vi "Tree_FocusArrayPath_Tests.vi"(11 "error in":errorcluster) -> (15 "error out":errorcluster)   [LabVIEW 2016, in "DronaTest.lvlib"]
uses:
  DronaTest.lvlib
  APIs/Stimulus/ControlValue/SetValueAuto.vi
  APIs/Stimulus/ControlValue/Controls/Tree/SetValueByHierarchicalPathArray.vi
  APIs/Assert/AssertControlValue/Controls/Tree/AssertValueByArrayPath.vi
  <vilib>/addons/_JKI Toolkits/Caraya/classes/Assert/Assert Error.vi
  <vilib>/addons/_JKI Toolkits/Caraya/classes/Assert/Assert Equal Value_Variant.vi
  <vilib>/addons/_JKI Toolkits/Caraya/classes/Test/Test.lvclass
  Drona.lvlib
  <vilib>/SLL Toolkit/SLL Debug/SLL Debug.lvlib
  <vilib>/addons/_JKI Toolkits/Caraya/classes/Assert/Assert.lvclass
  APIs/Stimulus/ControlValue/Controls/Tree/StimulusTree.lvlib
  APIs/Assert/AssertControlValue/Controls/Tree/AssertTree.lvlib
  APIs/Stimulus/ControlValue/ControlValue.lvlib
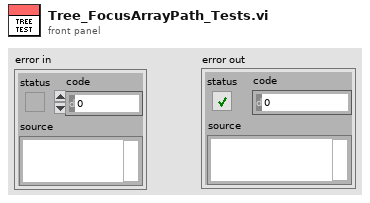
[diagram p1: front panel]
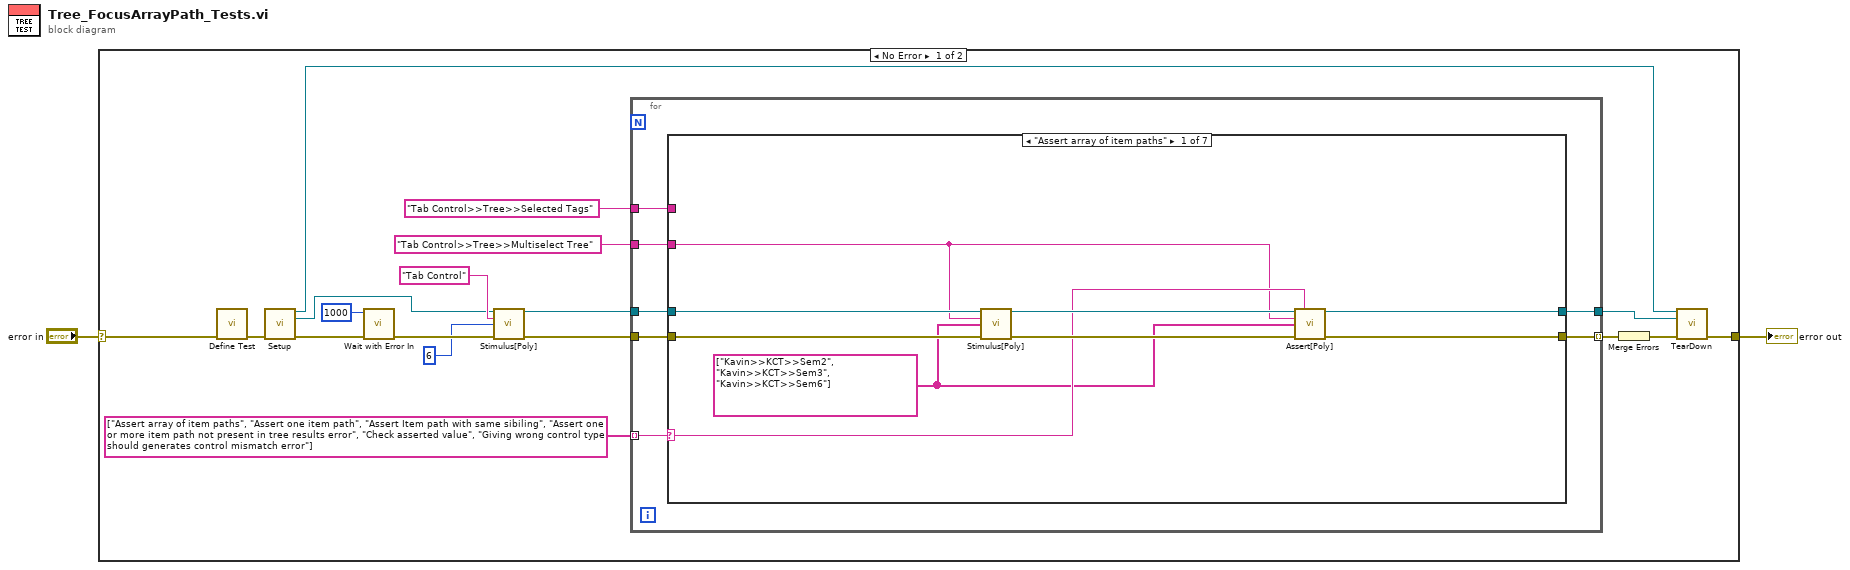
[diagram p0: block diagram]
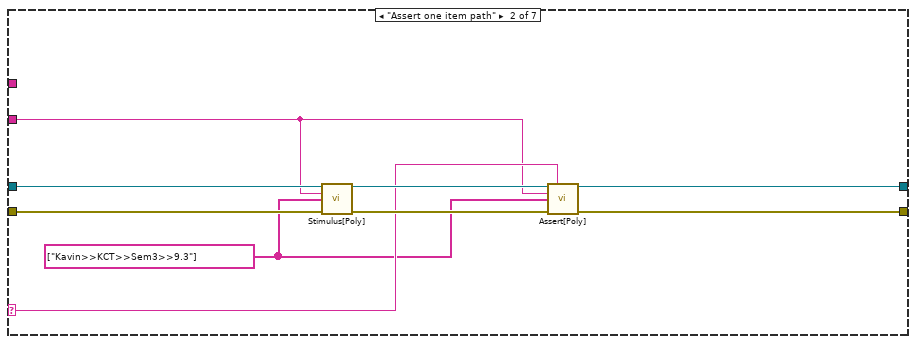
[diagram p2: hidden frame]
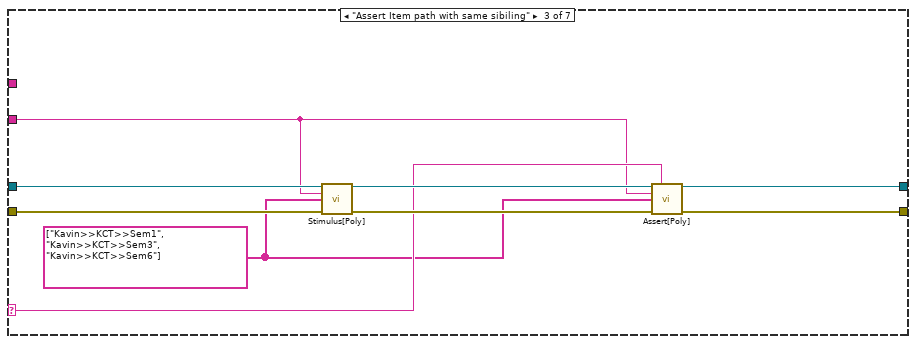
[diagram p3: hidden frame]
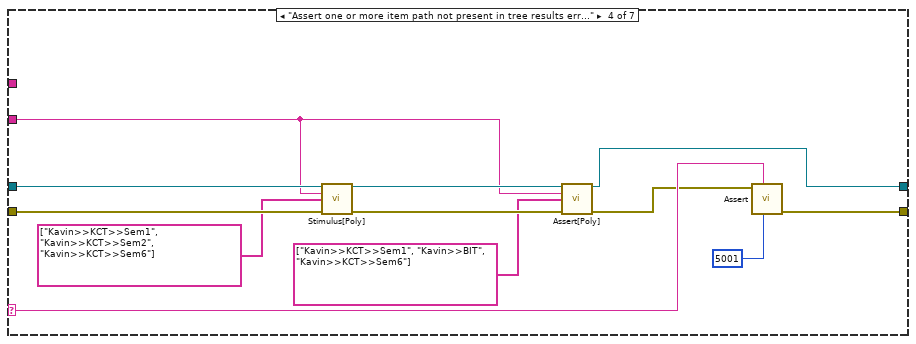
[diagram p4: hidden frame]
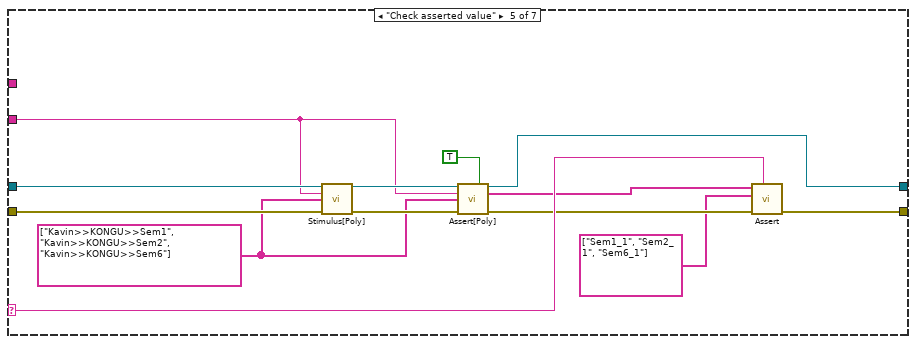
[diagram p5: hidden frame]
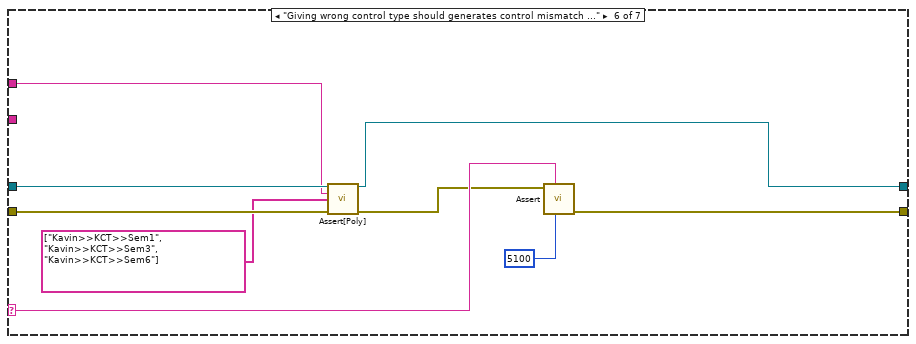
[diagram p6: hidden frame]
diagram:
  n1 = case shown="No Error" "error in" {
    selector: "error in" -> [w20 w91]
    tunnel: [w3 w91] -> w1
    frame No Error {
      n2 = call <vilib>:"Define Test.vi"("error in (no error)"=w20) -> ("error out"=w9:errorcluster)  [unwired: 9 in, 1 out]
      n3 = call "Setup.vi"("error in"=w9) -> ("Application Ref"=w4:refnum<vi>, "VI out"=w8:refnum<vi>, "error out"=w7:errorcluster)  [unwired: 12 in]
      n4 = call <vilib>:"Wait with Error In.vi"("error in (no error)"=w7, "milliseconds to wait"=u32 1000) -> ("error out"=w18:errorcluster)  [unwired: 9 in]
      n5 = call-poly "Stimulus[Poly].vi"("VI Reference In"=w8, "Control Path"="Tab Control", "Value (Signaling)"=6, "error in"=w18) -> ("VI Reference Out"=w14:refnum<vi>, "error out"=w17:errorcluster)  [unwired: 10 in]
      n6 = for {
        tunnel: w14 -> [w26]
        tunnel: "Tab Control>>Tree>>Multiselect Tree" ("Control Path") -> [w25]
        tunnel: "Tab Control>>Tree>>Selected Tags" ("Control Path") -> [w24]
        tunnel: string[] ["Assert array of item paths", "Assert one item path", "Assert Item path with same sibiling", "Assert one or more item path not present in tree results error", "Check asserted value", "Giving wrong control type should generates control mismatch error"] -> [w22] mode=indexing
        tunnel: [w21] -> w5
        tunnel: w17 -> [w27]
        tunnel: [w23] -> w10 mode=indexing
        n7 = case shown="\"Assert array of item paths\"" w22 {
          selector: w22 -> [w30 w39 w48 w63 w76 w87 _]
          tunnel: w27 -> [w36 w45 w54 w66 w79 w85 w90]
          tunnel: w26 -> [w35 w44 w53 w65 w78 w83 w89]
          tunnel: w25 -> [w29 w38 w47 w57 w73 _ _]
          tunnel: w24 -> [_ _ _ _ _ w82 _]
          tunnel: [w32 w41 w50 w64 w77 w88 w90] -> w23
          tunnel: [w31 w40 w49 w56 w72 w80 w89] -> w21
          frame "Assert array of item paths" {
            w28 = string[] ["Kavin>>KCT>>Sem2", "Kavin>>KCT>>Sem3", "Kavin>>KCT>>Sem6"] ("Hierarchical Path Array")
            n8 = call-poly "Stimulus[Poly].vi"("VI Reference In"=w35, "Control Path"=w29, "Hierarchical Path Array"=w28, "Error In"=w36) -> ("VI Reference Out"=w33:refnum<vi>, "Error Out"=w34:errorcluster)  [unwired: 10 in]
            n9 = call-poly "Assert[Poly].vi"("VI Reference In"=w33, "Test Label"=w30, "Control Path"=w29, "Focus Item Path"=w28, "Error In"=w34) -> ("VI Reference Out"=w31:refnum<vi>, "Error Out"=w32:errorcluster)  [unwired: 8 in, 1 out]
          }
          frame "Assert one item path" {
            w37 = string[] ["Kavin>>KCT>>Sem3>>9.3"] ("Item Name")
            n10 = call-poly "Stimulus[Poly].vi"("VI Reference In"=w44, "Control Path"=w38, "Hierarchical Path Array"=w37, "Error In"=w45) -> ("VI Reference Out"=w42:refnum<vi>, "Error Out"=w43:errorcluster)  [unwired: 10 in]
            n11 = call-poly "Assert[Poly].vi"("VI Reference In"=w42, "Test Label"=w39, "Control Path"=w38, "Focus Item Path"=w37, "Error In"=w43) -> ("VI Reference Out"=w40:refnum<vi>, "Error Out"=w41:errorcluster)  [unwired: 8 in, 1 out]
          }
          frame "Assert Item path with same sibiling" {
            w46 = string[] ["Kavin>>KCT>>Sem1", "Kavin>>KCT>>Sem3", "Kavin>>KCT>>Sem6"] ("Hierarchical Path Array")
            n12 = call-poly "Stimulus[Poly].vi"("VI Reference In"=w53, "Control Path"=w47, "Hierarchical Path Array"=w46, "Error In"=w54) -> ("VI Reference Out"=w51:refnum<vi>, "Error Out"=w52:errorcluster)  [unwired: 10 in]
            n13 = call-poly "Assert[Poly].vi"("VI Reference In"=w51, "Test Label"=w48, "Control Path"=w47, "Focus Item Path"=w46, "Error In"=w52) -> ("VI Reference Out"=w49:refnum<vi>, "Error Out"=w50:errorcluster)  [unwired: 8 in, 1 out]
          }
          frame "Assert one or more item path not present in tree results error" {
            n14 = call-poly "Stimulus[Poly].vi"("VI Reference In"=w65, "Control Path"=w57, "Hierarchical Path Array"=string[] ["Kavin>>KCT>>Sem1", "Kavin>>KCT>>Sem2", "Kavin>>KCT>>Sem6"], "Error In"=w66) -> ("VI Reference Out"=w58:refnum<vi>, "Error Out"=w60:errorcluster)  [unwired: 10 in]
            n15 = call-poly "Assert[Poly].vi"("VI Reference In"=w58, "Control Path"=w57, "Focus Item Path"=string[] ["Kavin>>KCT>>Sem1", "Kavin>>BIT", "Kavin>>KCT>>Sem6"] ("Hierarchical Path Array"), "Error In"=w60) -> ("VI Reference Out"=w56:refnum<vi>, "Error Out"=w59:errorcluster)  [unwired: 9 in, 1 out]
            n16 = call-poly <vilib>:"Assert.vi"("error code (1)"=5001, "Label"=w63, "Error?"=w59) -> ("error out"=w64:errorcluster)  [unwired: 7 in, 1 out]
          }
          frame "Check asserted value" {
            w71 = string[] ["Kavin>>KONGU>>Sem1", "Kavin>>KONGU>>Sem2", "Kavin>>KONGU>>Sem6"] ("Hierarchical Path Array")
            n17 = call-poly "Stimulus[Poly].vi"("VI Reference In"=w78, "Control Path"=w73, "Hierarchical Path Array"=w71, "Error In"=w79) -> ("VI Reference Out"=w74:refnum<vi>, "Error Out"=w75:errorcluster)  [unwired: 10 in]
            n18 = call-poly "Assert[Poly].vi"("VI Reference In"=w74, "Assert Only? (F)"=TRUE, "Control Path"=w73, "Focus Item Path"=w71, "Error In"=w75) -> ("VI Reference Out"=w72:refnum<vi>, "Asserted Value"=w68:string[], "Error Out"=w69:errorcluster)  [unwired: 8 in]
            n19 = call-poly <vilib>:"Assert.vi"("Label"=w76, "error in (no error)"=w69, "Y"=string[] ["Sem1_1", "Sem2_1", "Sem6_1"], "X"=w68) -> ("error out"=w77:errorcluster)  [unwired: 6 in, 1 out]
          }
          frame "Giving wrong control type should generates control mismatch error" {
            n20 = call-poly "Assert[Poly].vi"("VI Reference In"=w83, "Control Path"=w82, "Focus Item Path"=string[] ["Kavin>>KCT>>Sem1", "Kavin>>KCT>>Sem3", "Kavin>>KCT>>Sem6"] ("Hierarchical Path Array"), "Error In"=w85) -> ("VI Reference Out"=w80:refnum<vi>, "Error Out"=w84:errorcluster)  [unwired: 9 in, 1 out]
            n21 = call-poly <vilib>:"Assert.vi"("error code (1)"=5100, "Label"=w87, "Error?"=w84) -> ("error out"=w88:errorcluster)  [unwired: 7 in, 1 out]
          }
          frame Default {
          }
        }
      }
      n22 = Merge Errors(w10) -> (w6:errorcluster)
      n23 = call "TearDown.vi"("Application Ref"=w4, "VI in"=w5, "error in (no error)"=w6) -> ("error out"=w3:errorcluster)  [unwired: 12 in]
    }
    frame Error {
    }
  }
  "error out" <- w1
